vi "Check Action.vi"(6 "HRS Time":dbl, 7 "Values In":dbl[](array[numeric]), 8 "error in (no error)":errorcluster, 11 "Valve in":refnum<class "PeriodicControl.lvclass">) -> (0 "error out":errorcluster, 2 "Actions":T1[](array[typedef]), 3 "Valve out":refnum<class "PeriodicControl.lvclass">, 5 "Values":dbl[](array[numeric]))   [LabVIEW 2020, in "VolatusControl.lvlib" / "PeriodicControl.lvclass"]
uses:
  PeriodicControl.lvclass
  Control Action.ctl
  PeriodicControl.lvclass/PeriodicControl.ctl
  State.ctl
  Volatus/MessageQ/MessageQ.lvclass
  VolatusControl.lvlib
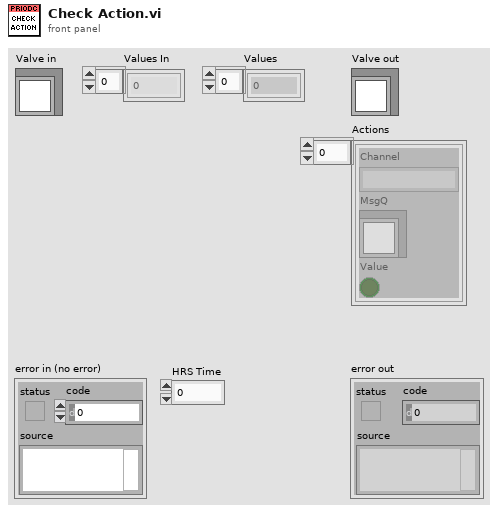
[diagram p1: front panel]
types:
  T1 = typedef "VolatusControl.lvlib/Control Action.ctl" = cluster{"Channel":string, "MsgQ":refnum<class "MessageQ.lvclass">, "Value":bool}
  T2 = typedef "VolatusControl.lvlib/PeriodicControl.lvclass/State.ctl" = enum16{"Idle", "Start", "Run", "Stop"}
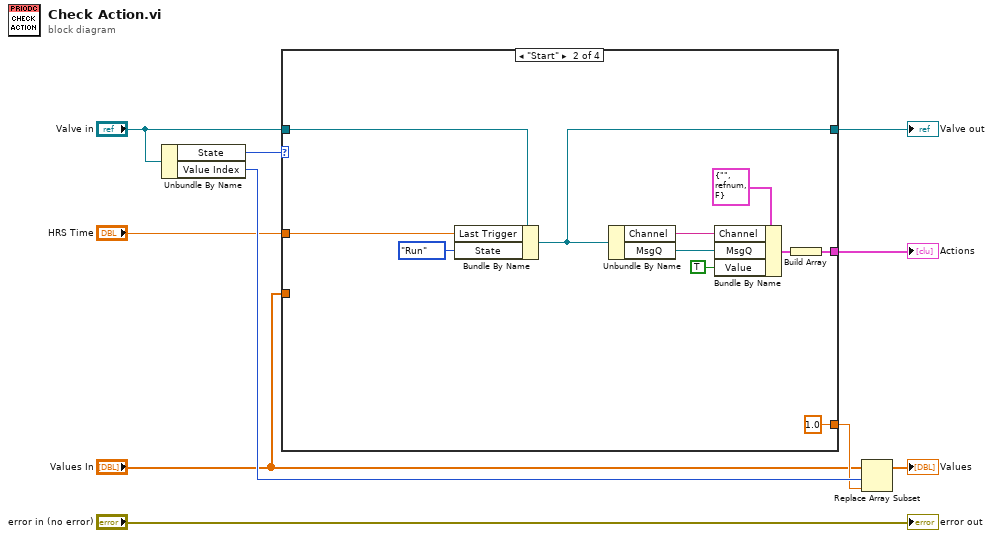
[diagram p0: block diagram]
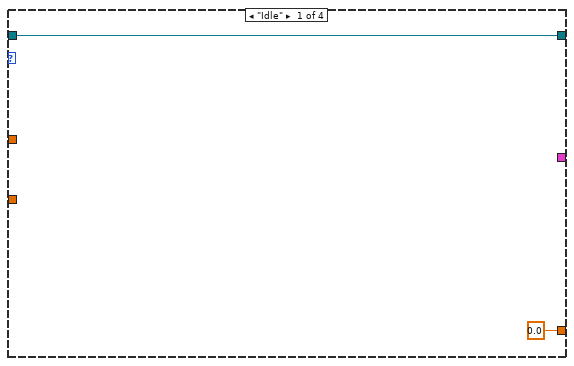
[diagram p2: hidden frame]
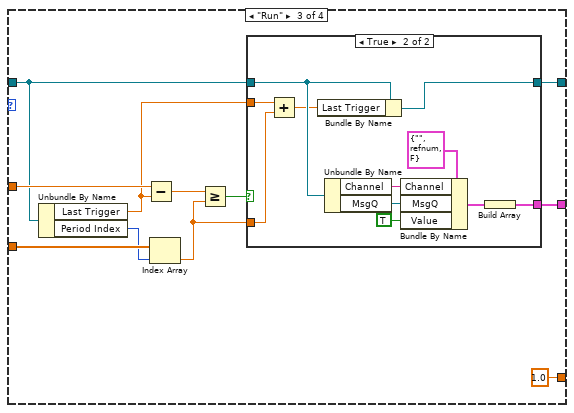
[diagram p3: hidden frame]
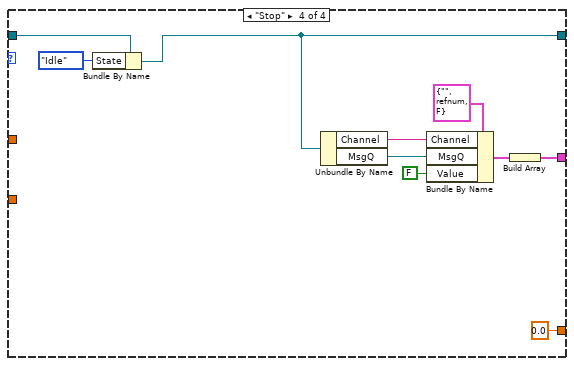
[diagram p5: hidden frame]
diagram:
  n1 = Unbundle By Name("Valve in") -> ("State"=w6:T2, "Value Index"=w8:i32)
  n2 = case shown="\"Start\"" w6 {
    tunnel: "Valve in" -> [w12 w18 w28 w50]
    tunnel: [w12 w17 w33 w48] -> w5
    tunnel: [0.0 1.0 1.0 0.0] -> w4
    tunnel: "HRS Time" -> [_ w16 w30 _]
    tunnel: [_ w13 w34 w47] -> w2
    tunnel: "Values In" -> [_ _ w32 _]
    frame "Idle" {
    }
    frame "Start" {
      n3 = Bundle By Name(cluster=w18, "Last Trigger"=w16, "State"=State."Run") -> (w17:refnum<class "PeriodicControl.lvclass">)
      n4 = Unbundle By Name(w17) -> ("Channel"=w20:string, "MsgQ"=w21:refnum<class "MessageQ.lvclass">)
      n5 = Bundle By Name(cluster=T1 {"Channel"="", "MsgQ"=refnum, "Value"=FALSE} ("Action"), "Channel"=w20, "MsgQ"=w21, "Value"=TRUE) -> (w22:T1)
      n6 = Build Array(w22) -> (w13:T1[])
    }
    frame "Run" {
      n7 = Unbundle By Name(w28) -> ("Last Trigger"=w25:dbl, "Period Index"=w31:i32)
      n8 = Subtract(x=w30, y=w25) -> (x-y=w29:dbl)
      n9 = Index Array(array=w32, index=w31) -> (element=w26:dbl)
      n10 = Greater Or Equal?(x=w29, y=w26) -> (x >= y?=w24:bool)
      n11 = case shown="True" w24 {
        tunnel: [_ w36] -> w34
        tunnel: w28 -> [w35 w40]
        tunnel: [w35 w41] -> w33
        tunnel: w26 -> [_ w38]
        tunnel: w25 -> [_ w39]
        frame False {
        }
        frame True {
          n12 = Add(x=w39, y=w38) -> (x+y=w37:dbl)
          n13 = Bundle By Name(cluster=w40, "Last Trigger"=w37) -> (w41:refnum<class "PeriodicControl.lvclass">)
          n14 = Unbundle By Name(w40) -> ("Channel"=w43:string, "MsgQ"=w44:refnum<class "MessageQ.lvclass">)
          n15 = Bundle By Name(cluster=T1 {"Channel"="", "MsgQ"=refnum, "Value"=FALSE} ("Action"), "Channel"=w43, "MsgQ"=w44, "Value"=TRUE) -> (w45:T1)
          n16 = Build Array(w45) -> (w36:T1[])
        }
      }
    }
    frame "Stop" {
      n17 = Bundle By Name(cluster=w50, "State"=State."Idle") -> (w48:refnum<class "PeriodicControl.lvclass">)
      n18 = Unbundle By Name(w48) -> ("Channel"=w53:string, "MsgQ"=w54:refnum<class "MessageQ.lvclass">)
      n19 = Bundle By Name(cluster=T1 {"Channel"="", "MsgQ"=refnum, "Value"=FALSE} ("Action"), "Channel"=w53, "MsgQ"=w54, "Value"=FALSE) -> (w51:T1)
      n20 = Build Array(w51) -> (w47:T1[])
    }
  }
  "Valve out" <- w5
  "Actions" <- w2
  n21 = Replace Array Subset(array="Values In", new element=w4, index=w8) -> (→"Values":dbl[])
  "error out" <- "error in (no error)"
